vi "LabApp - Make Table Report.vi"(5 "file params":T1={"path pattern"=enum."Y\\M\\D\\Tag.ext", "file extension (.bin)"=".bin"}, 6 "reverse order (F)":bool, 7 "log directory":path=path "DataLog", 9 "time range":cluster{"t1":dbl, "t2":dbl} {"t2" format="%<%H:%M:%S%2u\n%d/%m/%Y>T"; "t1" format="%<%H:%M:%S%2u\n%d/%m/%Y>T"}, 10 "Str Tags":string[](array[string]), 11 "Num Tags":string[](array[string])) -> (1 "Report Data":string[][](array[string]), 2 "Column Headers (Tags)":string[](array[string]), 3 "Row Headers (timestamps)":string[](array[string]))   [LabVIEW 2021]
doc: "::: CalcExpress Toolkit :::\nCopyright (c) 2000-2026 Konstantin Shifershteyn. All rights reserved."
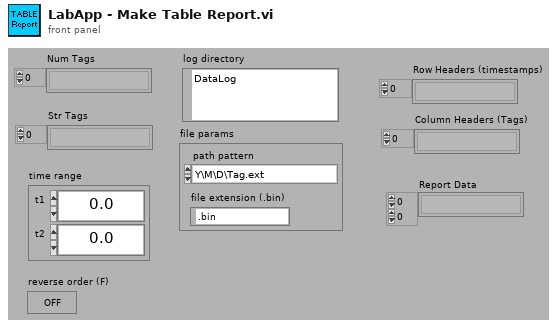
[diagram p1: front panel]
types:
  T1 = cluster{"path pattern":enum32{"Y\\M\\D\\Tag.ext", "Y\\M\\D\\Tag [Y-M-D].ext", "Y-M-D\\Tag.ext", "Y-M-D\\Tag [Y-M-D].ext", "Tag [Y-M-D].ext"}, "file extension (.bin)":string}
  T2 = cluster{"time stamps out":dbl[], "history data out":dbl[]}
  T3 = cluster{"max time stamp":dbl, "min time stamp":dbl, dbl}
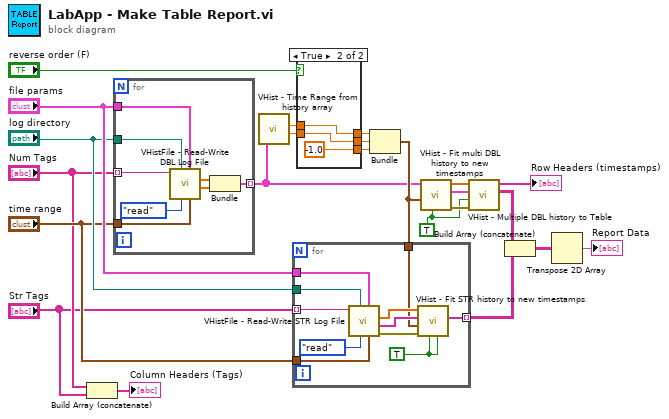
[diagram p0: block diagram]
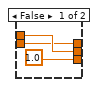
[diagram p2: hidden frame]
diagram:
  w3 = TRUE ("Interpolate (T)")
  n1 = Build Array (concatenate)("Num Tags", "Str Tags") -> (→"Column Headers (Tags)":string[])
  n2 = for {
    tunnel: [w29] -> w5 mode=indexing
    tunnel: "time range" -> [w28]
    tunnel: "log directory" -> [w27]
    tunnel: "Num Tags" -> [w25] mode=indexing
    tunnel: "file params" -> [w24]
    n3 = call "VHistFile - Read-Write DBL Log File.vi"("time range to read"=w28, "file params"=w24, "operation"=enum16{"nop", "read", "write"}."read", "log directory"=w27, "file tag"=w25) -> ("history data out"=w30:dbl[], "time stamps out"=w31:dbl[])  [unwired: 4 in, 1 out]
    n4 = Bundle("time stamps out"=w31, "history data out"=w30) -> (w29:T2)  [unwired: 1 in]
  }
  n5 = call "VHist - Time Range from history array.vi"("history array"=w5) -> ("max time stamp"=w2:dbl, "min time stamp"=w1:dbl)  [unwired: 4 in]
  n6 = case shown="True" "reverse order (F)" {
    tunnel: w2 -> [w34 w37]
    tunnel: [w33 w37] -> w9
    tunnel: [w34 w36] -> w8
    tunnel: w1 -> [w33 w36]
    tunnel: [1.0 -1.0] -> w7
    frame False {
    }
    frame True {
    }
  }
  n7 = Bundle("max time stamp"=w9, "min time stamp"=w8, w7) -> (w6:T3)  [unwired: 1 in]
  n8 = for {
    tunnel: "time range" -> [w48]
    tunnel: "log directory" -> [w47]
    tunnel: "Str Tags" -> [w45] mode=indexing
    tunnel: "file params" -> [w44]
    tunnel: w6 -> [w40]
    tunnel: [w39] -> w15 mode=indexing
    w38 = TRUE ("empty for absent (T)")
    n9 = call "VHistFile - Read-Write STR Log File.vi"("time range to read"=w48, "file params"=w44, "operation"=enum16{"nop", "read", "write"}."read", "log directory"=w47, "file tag"=w45) -> ("error out"=w43:errorcluster, "history data out"=w41:string[], "time stamps out"=w42:dbl[])  [unwired: 4 in]
    n10 = call "VHist - Fit STR history to new timestamps.vi"("merge data (T)"=w38, "empty for absent (T)"=w38, "error in"=w43, "time condition"=w40, "history data"=w41, "time stamps"=w42) -> ("history data out"=w39:string[])  [unwired: 3 in, 2 out]
  }
  n11 = call "VHist - Fit multi DBL history to new timestamps.vi"("NaN for absent (F)"=w3, "time condition"=w6, "history array"=w5) -> ("error out"=w23:errorcluster, "multiple history data out"=w22:cluster{"history data":dbl[]}[], "time stamps out"=w21:dbl[])  [unwired: 6 in]
  n12 = call "VHist - Multiple DBL history to Table.vi"("error in"=w23, "empty for NaN (F)"=w3, "multiple history data"=w22, "time stamps"=w21) -> ("table data"=w20:string[][], "time stamp headers"=→"Row Headers (timestamps)":string[])  [unwired: 5 in, 1 out]
  n13 = Build Array (concatenate)(w20, w15) -> (w19:string[][])
  n14 = Transpose 2D Array(2D array=w19) -> (transposed array=→"Report Data":string[][])
